vi "3.Open_Vi.vi"(8 "error in (no error)":errorcluster, 11 "VI Selection":T1=enum."Option window Vi") -> (0 "error out":errorcluster)   [LabVIEW 2021]
uses:
  Template/Main_VI/Control/Vi_selection.ctl
panel:
  out "error in (no error) 2":errorcluster
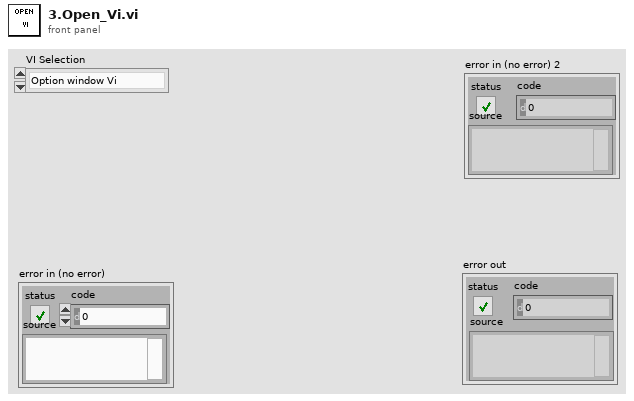
[diagram p1: front panel]
types:
  T1 = typedef "Vi_selection.ctl" = enum16{"Test Editor", "Option window Vi"}
  T2 = enum32{"Invalid", "Standard", "Closed", "Hidden", "Minimized", "Maximized"}
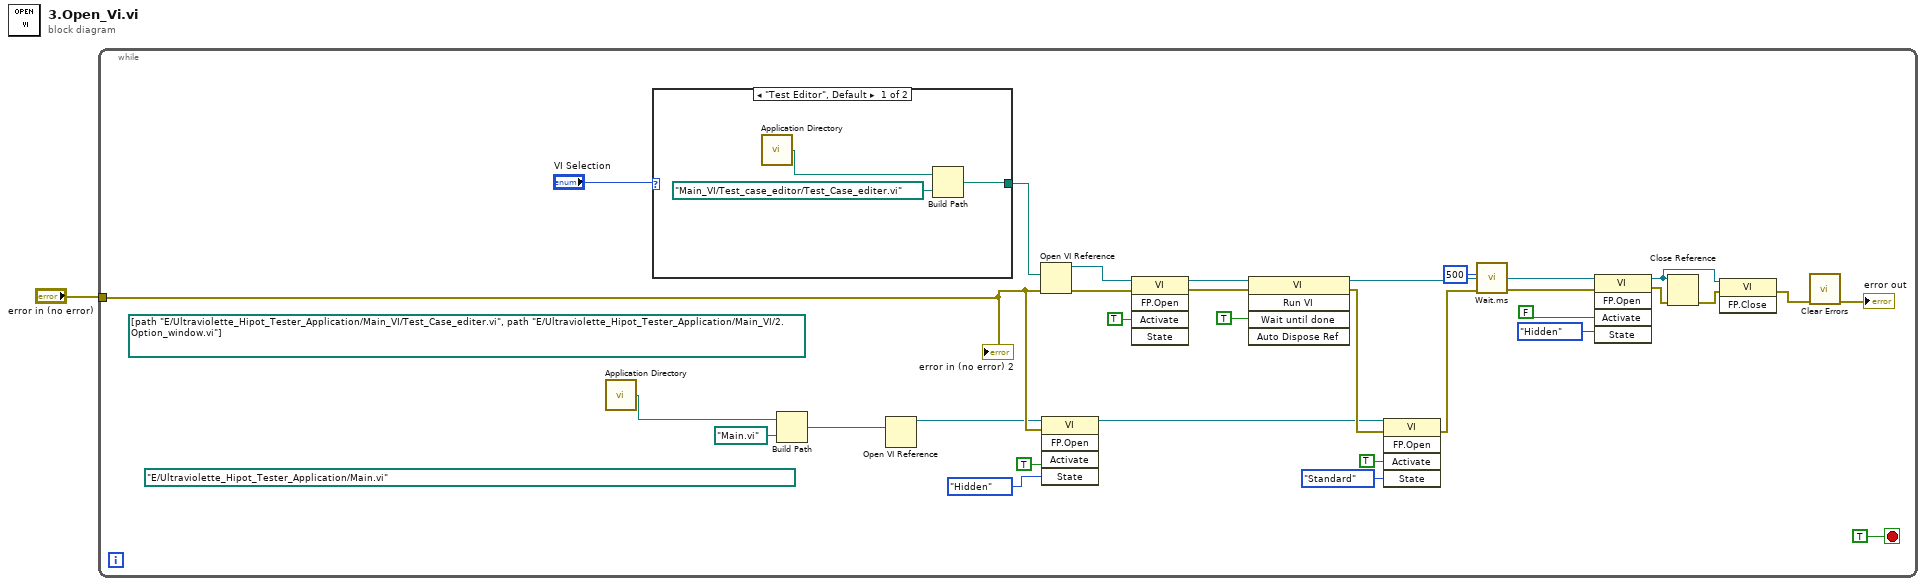
[diagram p0: block diagram]
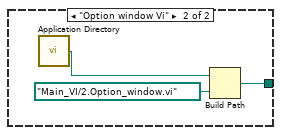
[diagram p2: hidden frame]
diagram:
  n1 = while {
    tunnel: "error in (no error)" -> [w13]
    stop <- TRUE stop-if-true
    (unwired) path "E:/Ultraviolette_Hipot_Tester_Application/Main.vi" ("vi path")
    (unwired) path[] [path "E:/Ultraviolette_Hipot_Tester_Application/Main_VI/Test_Case_editer.vi", path "E:/Ultraviolette_Hipot_Tester_Application/Main_VI/2.Option_window.vi"]
    n2 = call <vilib>:"Application Directory.vi"() -> ("Application Directory"=w3:path)
    n3 = case shown="\"Test Editor\", Default" "VI Selection" {
      tunnel: [w33 w36] -> w5
      frame "Test Editor", Default {
        n4 = call <vilib>:"Application Directory.vi"() -> ("Application Directory"=w35:path)
        n5 = Build Path(base path=w35, name or relative path=path "Main_VI/Test_case_editor/Test_Case_editer.vi") -> (appended path=w33:path)
      }
      frame "Option window Vi" {
        n6 = call <vilib>:"Application Directory.vi"() -> ("Application Directory"=w38:path)
        n7 = Build Path(base path=w38, name or relative path=path "Main_VI/2.Option_window.vi") -> (appended path=w36:path)
      }
    }
    n8 = Build Path(base path=w3, name or relative path=path "Main.vi") -> (appended path=w2:path)
    n9 = Open VI Reference(vi path=w2) -> (vi reference=w10:refnum<vi>)  [unwired: 5 in, 1 out]
    n10 = Open VI Reference(vi path=w5, error in (no error)=w13) -> (vi reference=w30:refnum<vi>, error out=w26:errorcluster)  [unwired: 4 in]
    n11 = invoke class="VI" method="FP.Open"(reference=w10, error in=w13, "Activate"=TRUE ("Activate?"), "State"=T2."Hidden") -> (reference out=w7:refnum<vi>)  [unwired: 1 in, 4 out]
    n12 = invoke class="VI" method="FP.Open"(reference=w30, error in=w26, "Activate"=TRUE ("Activate?")) -> (reference out=w28:refnum<vi>, error out=w27:errorcluster)  [unwired: 2 in, 3 out]
    n13 = invoke class="VI" method="Run VI"(reference=w28, error in=w27, "Wait until done"=TRUE ("Wait Until Done")) -> (reference out=w25:refnum<vi>, error out=w21:errorcluster)  [unwired: 2 in, 3 out]
    n14 = invoke class="VI" method="FP.Open"(reference=w7, error in=w21, "Activate"=TRUE ("Activate?"), "State"=T2."Standard") -> (error out=w19:errorcluster)  [unwired: 1 in, 4 out]
    n15 = call "Wait.ms.vi"("error in"=w19, "milliseconds to wait"=u32 500) -> ("error out"=w20:errorcluster)  [unwired: 9 in]
    n16 = invoke class="VI" method="FP.Open"(reference=w25, error in=w20, "Activate"=FALSE ("Activate?"), "State"=T2."Hidden") -> (reference out=w15:refnum<vi>, error out=w24:errorcluster)  [unwired: 1 in, 3 out]
    n17 = Close Reference(reference=w15, error in (no error)=w24) -> (error out=w16:errorcluster)
    n18 = invoke class="VI" method="FP.Close"(reference=w15, error in=w16) -> (error out=w17:errorcluster)  [unwired: 1 in, 2 out]
    n19 = call <vilib>:"Clear Errors.vi"("error in (no error)"=w17) -> ("error out"=→"error out":errorcluster)  [unwired: 5 in, 1 out]
    "error in (no error) 2" <- w13
  }
